vi "Create Raw Reader.vi"(6 "Timeout (ms)":u32=5000, 8 "error in (no error)":errorcluster, 10 "Topic Full Names":T1) -> (0 "error out":errorcluster, 3 "Raw Reader Reference":T2 {"refnum" format="%.0x"})   [LabVIEW 2021, in "Iceoryx.lvlib"]
uses:
  Iceoryx.lvlib
  typedef/Topic Full Names.ctl
  typedef/Errors.ctl
  SubVIs/Add Error Core.vi
  <vilib>/CIF Foundation/CIF Utilities/File/SubVIs/File Not Found Error Core.vi
  SubVIs/Convert Error Core.vi
  <vilib>/CIF Foundation/CIF Utilities/File/File_CIF_U.lvlib
  Refnum/Typedef/BB Raw Reader Refnum.ctl
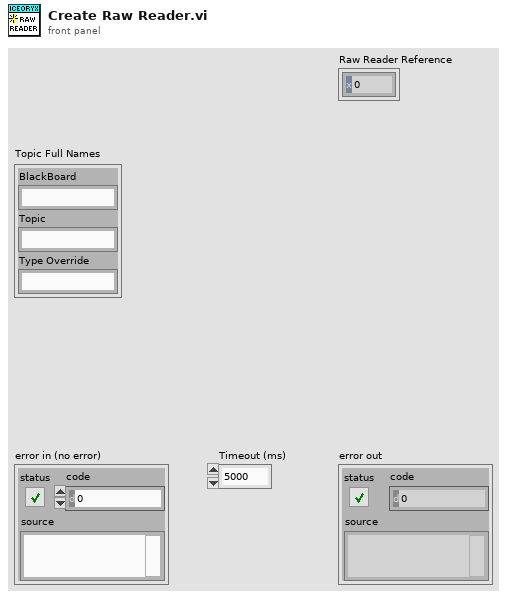
[diagram p1: front panel]
types:
  T1 = typedef "Iceoryx.lvlib/Topic Full Names.ctl" = cluster{"BlackBoard":string, "Topic":string, "Type Override":string}
  T2 = typedef "Iceoryx.lvlib/BB Raw Reader Refnum.ctl" = cluster{"refnum":u64, "BB Raw Reader":enum8{"bb_raw_reader"}}
  T3 = typedef "Iceoryx.lvlib/Errors.ctl" = enum16{"Unsupported Type", "Empty Name", "Cluster Name"}
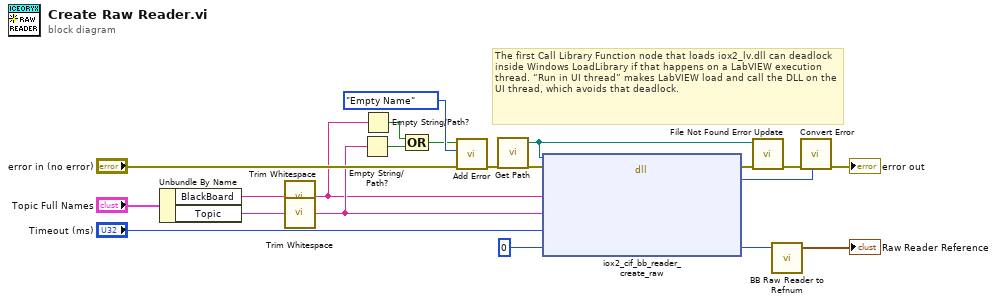
[diagram p0: block diagram]
diagram:
  # "The first Call Library Function node that loads iox2_lv.dll can deadlock inside Windows LoadLibrary if that happens on a LabVIEW execution thread. “Run in UI thread” makes LabVIEW load and call the DLL on the UI thread, which avoids that deadlock."
  n1 = Unbundle By Name("Topic Full Names") -> ("BlackBoard"=w4:string, "Topic"=w3:string)
  n2 = call <vilib>:"Trim Whitespace.vi"("string"=w4) -> ("trimmed string"=w6:string)  [unwired: 1 in]
  n3 = call <vilib>:"Trim Whitespace.vi"("string"=w3) -> ("trimmed string"=w7:string)  [unwired: 1 in]
  n4 = Empty String/Path?(string/path=w7) -> (empty?=w10:bool)
  n5 = Empty String/Path?(string/path=w6) -> (empty?=w9:bool)
  n6 = Compound Arithmetic op=OR(w9, w10) -> (w8:bool)
  n7 = call "Add Error.vi"("error in (no error)"="error in (no error)", "Error"=Errors."Empty Name", "Insert Error"=w8) -> ("error out"=w2:errorcluster)  [unwired: 8 in]
  n8 = call "Get Path.vi"() -> ("libiox2_cif path"=w16:path)  [unwired: 4 in]
  n9 = dll-call lib="D:/dev/iceoryx2_lvwrapper/dist/iox2_cif.dll" fn="iox2_cif_bb_reader_create_raw"(path in=w16, error in=w2, "bb_name"=w6, "topic"=w7, "timeout_ms"="Timeout (ms)", "reader"=u64 0 ("writer")) -> (error out=w15:errorcluster, "return type"=w14:i32, "reader"=w20:u64)  [unwired: 4 in, 1 out]
  n10 = call <vilib>:"File Not Found Error Update.vi"("error in"=w15, "path in"=w16) -> ("error out"=w17:errorcluster)  [unwired: 9 in]
  n11 = call "BB Raw Reader to Refnum.vi"("BB Raw Reader U64"=w20) -> ("BB Raw Reader Refnum"=→"Raw Reader Reference":T2)  [unwired: 4 in]
  n12 = call "Convert Error.vi"("return type"=w14, "error in (no error)"=w17) -> ("error out"=→"error out":errorcluster)  [unwired: 9 in]
